vi "Set Tunnel Flags.vi"(8 "error in (no error)":errorcluster, 11 "Struct Refnum":refnum<vi>) -> (0 "error out":errorcluster, 3 "reference out":refnum<vi>)   [LabVIEW 2012, in "Scripting Tools.lvlib"]
uses:
  Scripting Tools.lvlib
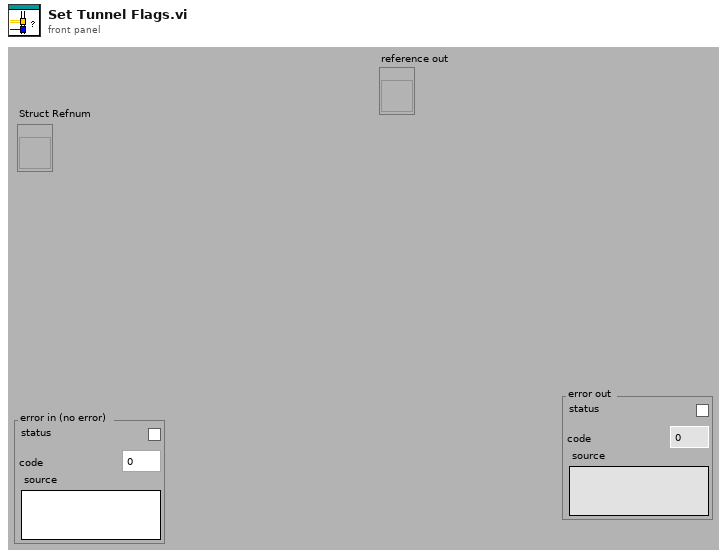
[diagram p1: front panel]
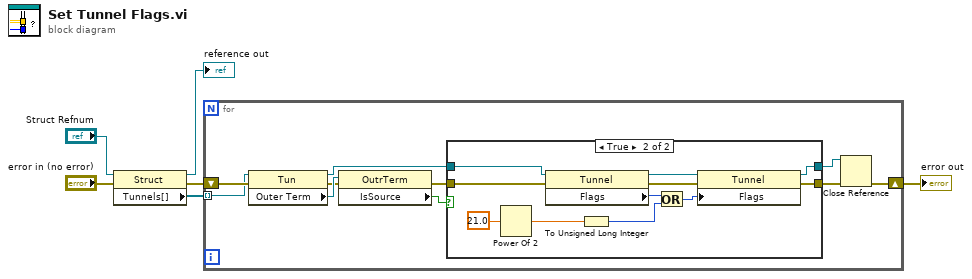
[diagram p0: block diagram]
diagram:
  n1 = property class="Struct"(reference="Struct Refnum", error in="error in (no error)") -> (reference out=→"reference out":refnum<vi>, error out=w3:errorcluster, "Tunnels[]"=w4:refnum<vi>[])
  n2 = for {
    tunnel: w4 -> [w15] mode=indexing
    shift-right: [w8] -> w1
    shift-left: w3 -> [w16]
    n3 = property class="Tun"(reference=w15, error in=w16) -> (reference out=w12:refnum<vi>, error out=w13:errorcluster, "Outer Term"=w14:refnum<vi>)
    n4 = property class="OutrTerm"(reference=w14, error in=w13) -> (error out=w11:errorcluster, "IsSource"=w9:bool)  [unwired: 1 out]
    n5 = case shown="True" w9 {
      tunnel: w12 -> [w17 w29]
      tunnel: w11 -> [w18 w28]
      tunnel: [w18 w23] -> w10
      tunnel: [w17 w22] -> w7
      frame False {
      }
      frame True {
        n6 = Power Of 2(x=21.0) -> (2^x=w21:dbl)
        n7 = property class="Tunnel"(reference=w29, error in=w28) -> (reference out=w26:refnum<vi>, error out=w27:errorcluster, "Flags"=w25:u32)
        n8 = To Unsigned Long Integer(number=w21) -> (unsigned 32bit integer=w20:u32)
        n9 = Or(x=w25, y=w20) -> (x .or. y?=w24:u32)
        n10 = property class="Tunnel"(reference=w26, error in=w27, "Flags"=w24) -> (reference out=w22:refnum<vi>, error out=w23:errorcluster)
      }
    }
    n11 = Close Reference(reference=w7, error in (no error)=w10) -> (error out=w8:errorcluster)
  }
  "error out" <- w1
